vi "var to string (path).vi"(10 "Path":path, 11 "reference":refnum<vi>) -> (3 "path string":string)   [LabVIEW 2025]
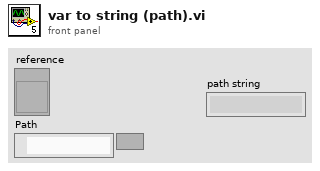
[diagram p1: front panel]
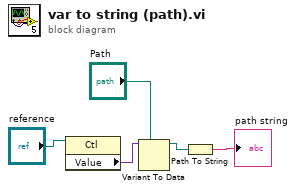
[diagram p0: block diagram]
diagram:
  n1 = property class="Ctl"(reference="reference") -> ("Value"=w5:variant)  [unwired: 1 in, 2 out]
  n2 = Variant To Data(type="Path", Variant=w5) -> (data=w2:path)  [unwired: 1 in, 1 out]
  n3 = Path To String(path=w2) -> (string=→"path string":string)
